vi "Reserve Sessions with Observer.vi"(6 "timeout (ms)":i32, 7 "reservation observer":refnum<class "IReservation Observer.lvclass">, 8 "error in":errorcluster, 9 "instrument type id":string, 10 "pin or relay names":string[](array[string]), 11 "pin map context":T1) -> (0 "error out":errorcluster, 3 "session reservation out":refnum<class "Session Reservation.lvclass">)   [LabVIEW 2021, in "NI Session Management V1 Client.lvlib" / "Session Reservation.lvclass"]
doc: "Reserves session(s) based on the provided instrument type and pin or its group information."
uses:
  Session Reservation.lvclass
  Session Reservation.lvclass/Session Reservation.ctl
  gRPC/Generated APIs/ni/measurementlink/sessionmanagement/v1/RPC Messages/ni_measurementlink_sessionmanagement_v1_ReserveSessionsRequest.ctl
  gRPC/Generated APIs/ni/measurementlink/sessionmanagement/v1/ni.measurementlink.sessionmanagement.v1.api.lvlib
  gRPC/Generated APIs/ni/measurementlink/sessionmanagement/v1/RPC Messages/ni_measurementlink_PinMapContext.ctl
  gRPC/Generated APIs/ni/measurementlink/sessionmanagement/v1/RPC Messages/ni_measurementlink_sessionmanagement_v1_ReserveSessionsRequest_AnnotationsEntry.ctl
  707f5494-25d6-43e3-965d-4bb78dbc0dc9.vi
  IReservation Observer/IReservation Observer.lvclass
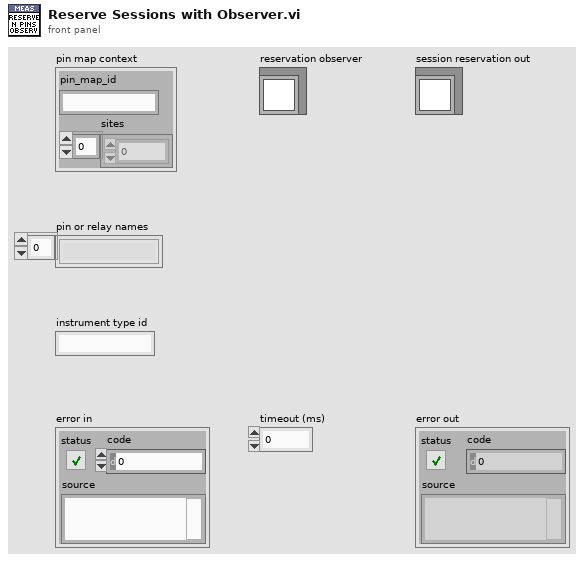
[diagram p1: front panel]
types:
  T1 = typedef "ni.measurementlink.sessionmanagement.v1.api.lvlib/ni_measurementlink_PinMapContext.ctl" = cluster{"pin_map_id":string, "sites":i32[]}
  T2 = typedef "ni.measurementlink.sessionmanagement.v1.api.lvlib/ni_measurementlink_sessionmanagement_v1_ReserveSessionsRequest_AnnotationsEntry.ctl" = cluster{"key":string, "value":string}
  T3 = typedef "ni.measurementlink.sessionmanagement.v1.api.lvlib/ni_measurementlink_sessionmanagement_v1_ReserveSessionsRequest.ctl" = cluster{"pin_map_context":T1, "pin_or_relay_names":string[], "instrument_type_id":string, "timeout_in_milliseconds":i32, "annotations":T2[]}
  T4 = typedef "ni.measurementlink.sessionmanagement.v1.api.lvlib/ni_measurementlink_sessionmanagement_v1_ReserveSessionsResponse.ctl" = cluster{"sessions":T5[], "multiplexer_sessions":T9[], "group_mappings":T11[]}
  T5 = typedef "ni.measurementlink.sessionmanagement.v1.api.lvlib/ni_measurementlink_sessionmanagement_v1_SessionInformation.ctl" = cluster{"session":T6, "resource_name":string, "channel_list":string, "instrument_type_id":string, "session_exists":bool, "session_reserved":bool, "channel_mappings":T7[], "annotations":T8[]}
  T6 = typedef "ni.measurementlink.sessionmanagement.v1.api.lvlib/nidevice_grpc_Session.ctl" = cluster{"name":string}
  T7 = typedef "ni.measurementlink.sessionmanagement.v1.api.lvlib/ni_measurementlink_sessionmanagement_v1_ChannelMapping.ctl" = cluster{"pin_or_relay_name":string, "site":i32, "channel":string, "multiplexer_resource_name":string, "multiplexer_route":string}
  T8 = typedef "ni.measurementlink.sessionmanagement.v1.api.lvlib/ni_measurementlink_sessionmanagement_v1_SessionInformation_AnnotationsEntry.ctl" = cluster{"key":string, "value":string}
  T9 = typedef "ni.measurementlink.sessionmanagement.v1.api.lvlib/ni_measurementlink_sessionmanagement_v1_MultiplexerSessionInformation.ctl" = cluster{"session":T6, "resource_name":string, "multiplexer_type_id":string, "session_exists":bool, "annotations":T10[]}
  T10 = typedef "ni.measurementlink.sessionmanagement.v1.api.lvlib/ni_measurementlink_sessionmanagement_v1_MultiplexerSessionInformation_AnnotationsEntry.ctl" = cluster{"key":string, "value":string}
  T11 = typedef "ni.measurementlink.sessionmanagement.v1.api.lvlib/ni_measurementlink_sessionmanagement_v1_ReserveSessionsResponse_GroupMappingsEntry.ctl" = cluster{"key":string, "value":T12}
  T12 = typedef "ni.measurementlink.sessionmanagement.v1.api.lvlib/ni_measurementlink_sessionmanagement_v1_ResolvedPinsOrRelays.ctl" = cluster{"pin_or_relay_names":string[]}
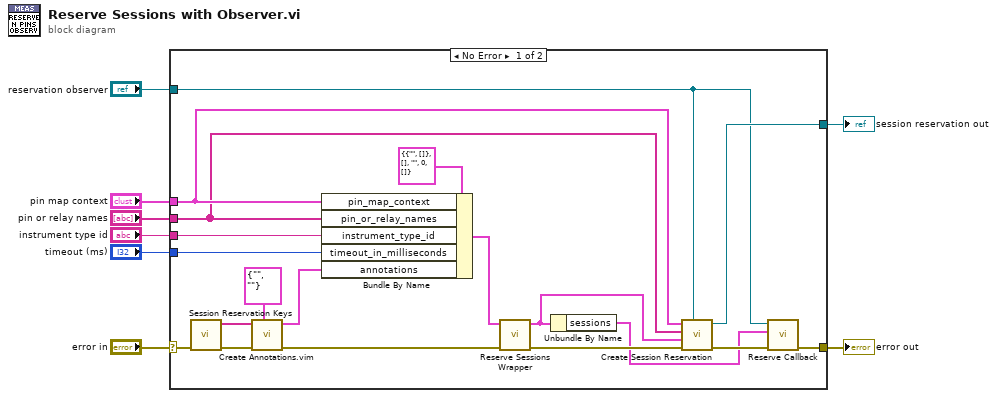
[diagram p0: block diagram]
diagram:
  n1 = case shown="No Error" "error in" {
    selector: "error in" -> [w16 w27]
    tunnel: "instrument type id" -> [w26 _]
    tunnel: "pin or relay names" -> [w22 _]
    tunnel: "pin map context" -> [w23 _]
    tunnel: [w20 w27] -> w5
    tunnel: [w24 _] -> w4
    tunnel: "reservation observer" -> [w19 _]
    tunnel: "timeout (ms)" -> [w13 _]
    frame No Error {
      n2 = call "Session Reservation Keys.vi"() -> ("reserve annotation keys"=w12:string[])  [unwired: 11 in]
      n3 = call "Create Annotations.vim"("annotation typedef"=T2 {"key"="", "value"=""} ("ni_measurementlink_sessionmanagement_v1_ReserveSessionsRequest_AnnotationsEntry"), "error in"=w16, "annotation keys"=w12) -> ("error out"=w14:errorcluster, "annotations array"=w10:T2[])  [unwired: 7 in]
      n4 = Bundle By Name(cluster=T3 {"pin_map_context"={"pin_map_id"="", "sites"=[]}, "pin_or_relay_names"=[], "instrument_type_id"="", "timeout_in_milliseconds"=0, "annotations"=[]} ("Request Data"), "pin_map_context"=w23, "pin_or_relay_names"=w22, "instrument_type_id"=w26, "timeout_in_milliseconds"=w13, "annotations"=w10) -> (w17:T3)
      n5 = call "Reserve Sessions Wrapper.vi"("error in"=w14, "request data"=w17) -> ("error out"=w25:errorcluster, "response data"=w15:T4)  [unwired: 8 in]
      n6 = Unbundle By Name(w15) -> ("sessions"=w18:T5[])
      n7 = call "Create Session Reservation.vi"("reservation observer"=w19, "error in"=w25, "session reservation response"=w15, "pin or relay names"=w22, "pin map context"=w23) -> ("error out"=w21:errorcluster, "session reservation out"=w24:refnum<class "Session Reservation.lvclass">)  [unwired: 5 in]
      n8 = call-dynamic "Reserve Callback.vi"("error in"=w21, "session infos"=w18, "reservation observer in"=w19) -> ("error out"=w20:errorcluster)  [unwired: 7 in, 1 out]
    }
    frame Error {
    }
  }
  "session reservation out" <- w4
  "error out" <- w5
